vi "Get All NI-SWITCH Properties.vi"(8 "error in":errorcluster, 11 "ni-switch custom device in":T2 format="%.0x") -> (0 "error out":errorcluster, 2 "properties":T1, 3 "ni-switch custom device out":T2 format="%.0x")   [LabVIEW 2020, in "NI-SWITCH Scripting.lvlib"]
uses:
  NI-SWITCH Scripting.lvlib
  <vilib>/NI VeriStand/Custom Device API/Custom Device Item Ref.ctl
  NI-SWITCH All Properties.ctl
  <vilib>/NI VeriStand/Custom Device API/Custom Device API.lvlib
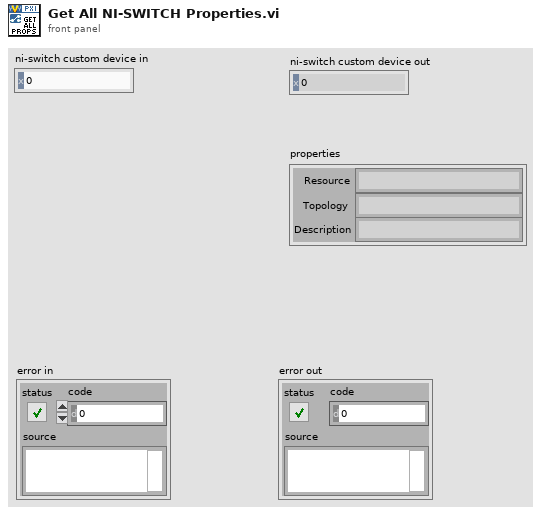
[diagram p1: front panel]
types:
  T1 = typedef "NI-SWITCH Scripting.lvlib/NI-SWITCH All Properties.ctl" = cluster{"Resource":string, "Topology":string, "Description":string}
  T2 = typedef "Custom Device API.lvlib/Custom Device Item Ref.ctl" = u64
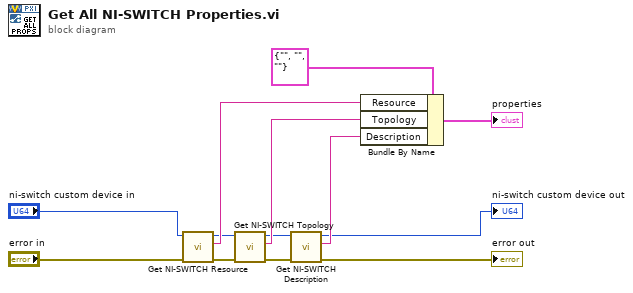
[diagram p0: block diagram]
diagram:
  n1 = call "Get NI-SWITCH Resource.vi"("error in"="error in", "ni-switch custom device in"="ni-switch custom device in") -> ("error out"=w5:errorcluster, "resource"=w10:string, "ni-switch custom device out"=w6:T2)  [unwired: 7 in]
  n2 = call "Get NI-SWITCH Topology.vi"("error in"=w5, "ni-switch custom device in"=w6) -> ("error out"=w1:errorcluster, "topology"=w9:string, "ni-switch custom device out"=w2:T2)  [unwired: 7 in]
  n3 = call "Get NI-SWITCH Description.vi"("error in"=w1, "ni-switch custom device in"=w2) -> ("error out"=→"error out":errorcluster, "description"=w7:string, "ni-switch custom device out"=→"ni-switch custom device out":T2)  [unwired: 7 in]
  n4 = Bundle By Name(cluster=T1 {"Resource"="", "Topology"="", "Description"=""} ("SLSC Switch All Properties"), "Resource"=w10, "Topology"=w9, "Description"=w7) -> (→"properties":T1)
